vi "Get TurnTable Angle.vi"(8 "error in (no error)":errorcluster caption="에러 입력(에러 없음)", 11 "Instrument Manager 입력":refnum<class "Instrument Manager.lvclass">) -> (0 "error out":errorcluster caption="에러 출력", 3 "Instrument Manager 출력":refnum<class "Instrument Manager.lvclass">)   [LabVIEW 2023, in "Instrument Manager.lvclass"]
uses:
  Instrument Manager.lvclass
  Instrument Manager.lvclass/Instrument Manager.ctl
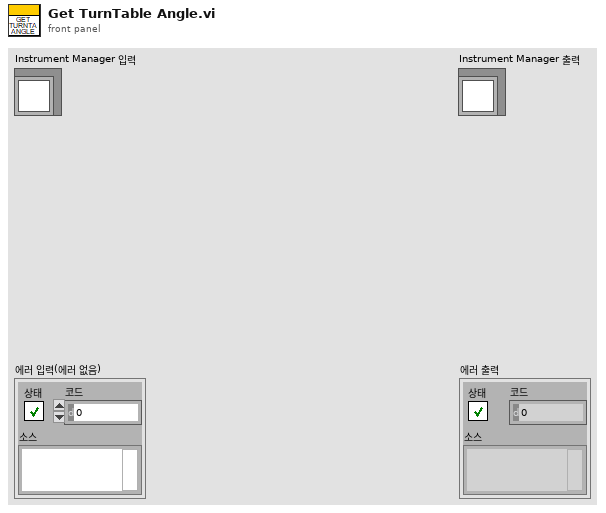
[diagram p1: front panel]
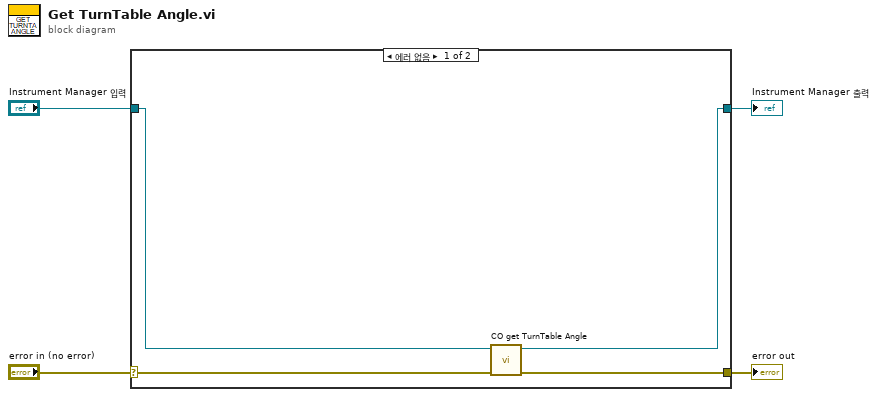
[diagram p0: block diagram]
diagram:
  n1 = case shown="에러 없음" "error in (no error)" {
    selector: "error in (no error)" -> [w8 w10]
    tunnel: [w7 w10] -> w3
    tunnel: [w5 w9] -> w1
    tunnel: "Instrument Manager 입력" -> [w6 w9]
    frame No Error {
      n2 = call "CO get TurnTable Angle.vi"("error in (no error)"=w8, "Instrument Manager 입력"=w6) -> ("error out"=w7:errorcluster, "Instrument Manager 출력"=w5:refnum<class "Instrument Manager.lvclass">)  [unwired: 7 in, 1 out]
    }
    frame Error {
    }
  }
  "error out" <- w3
  "Instrument Manager 출력" <- w1
